vi "VIH - CHM Project - Write TOC File - Add LabVIEW Files.vi"(7 "Base Dir Path":path, 8 "error in":errorcluster, 9 "Project Files":T2, 11 "HTML in":string) -> (0 "error out":errorcluster, 3 "HTML out":string)   [LabVIEW 2014]
doc: "::: VI Helpeks :::\nCopyright (c) 2000-2026 Konstantin Shifershteyn. All rights reserved."
uses:
  _VIH HelpGen - Palette.llb/VIH HelpGen Typedef - Palette - Item Type Enum.ctl
panel:
  # "VI Helpeks\nCopyright (c) 2012-2026 Konstantin Shifershteyn"
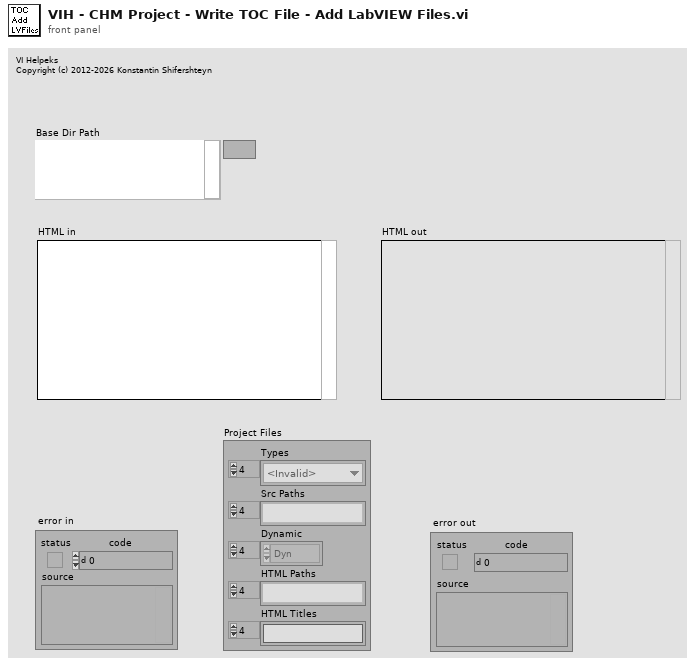
[diagram p1: front panel]
types:
  T1 = typedef "VIH HelpGen Typedef - Palette - Item Type Enum.ctl" = enum32{"<Invalid>", "<unknown>", "VI", "Menu", "LV Func", "Express VI", "Poly VI", "CTL", "HTML"}
  T2 = cluster{"Types":T1[], "Src Paths":path[], "Dynamic":enum16{"Dyn", "Stat", "Both"}[], "HTML Paths":path[], "HTML Titles":string[]}
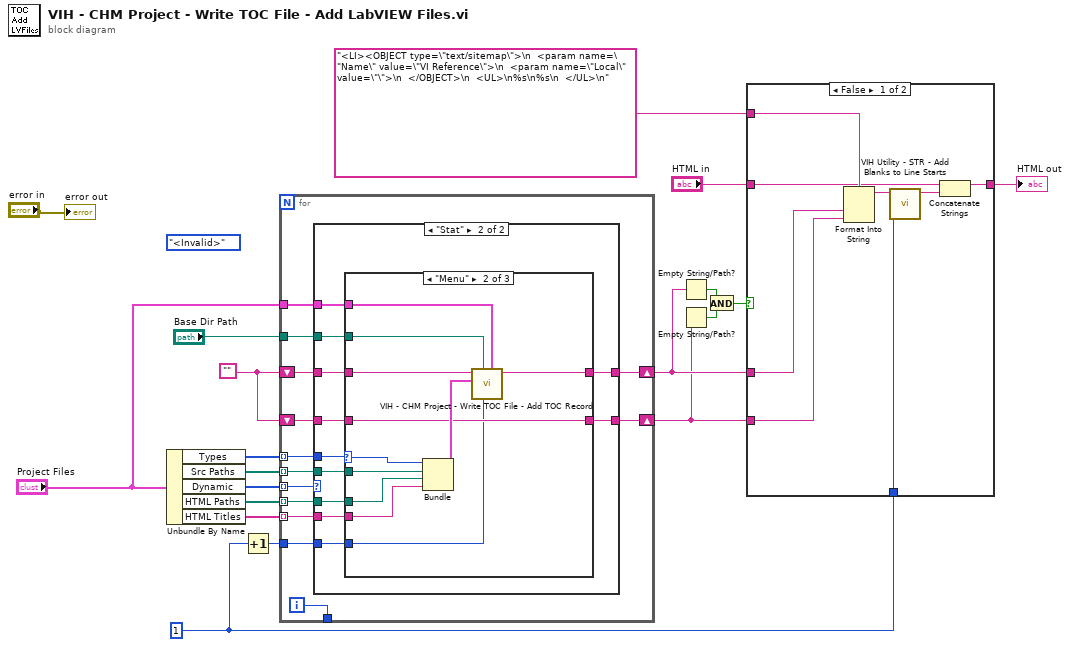
[diagram p0: block diagram]
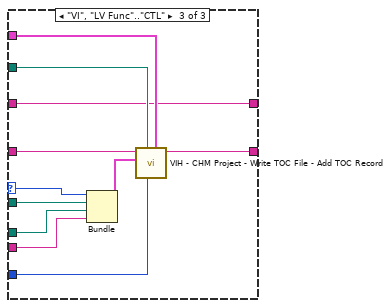
[diagram p5: hidden frame]
diagram:
  w2 = 1
  (unwired) VIH_HelpGen_Typedef_-_Palette_-_Item_Type_Enum."<Invalid>" ("Item/File Type")
  w11 = ""
  n1 = Unbundle By Name("Project Files") -> ("Types"=w17:T1[], "Src Paths"=w18:path[], "Dynamic"=w19:enum16{"Dyn", "Stat", "Both"}[], "HTML Paths"=w16:path[], "HTML Titles"=w14:string[])
  n2 = Increment(x=w2) -> (x+1=w1:i32)
  n3 = for {
    tunnel: w19 -> [w32] mode=indexing
    shift-right: [w29] -> w5
    shift-left: w11 -> [w31]
    tunnel: "Project Files" -> [w30]
    tunnel: w18 -> [w28] mode=indexing
    tunnel: w17 -> [w27] mode=indexing
    tunnel: w16 -> [w26] mode=indexing
    tunnel: "Base Dir Path" -> [w25]
    tunnel: w14 -> [w24] mode=indexing
    shift-right: [w22] -> w3
    shift-left: w11 -> [w23]
    tunnel: [w21] -> _
    tunnel: w1 -> [w20]
    i -> [w21]
    n4 = case shown="\"Stat\"" w32 {
      tunnel: w31 -> [w34 w45]
      tunnel: w30 -> [_ w44]
      tunnel: [w34 w43] -> w29
      tunnel: w28 -> [_ w41]
      tunnel: w27 -> [_ w38]
      tunnel: w26 -> [_ w40]
      tunnel: w25 -> [_ w42]
      tunnel: w24 -> [_ w39]
      tunnel: w23 -> [w33 w37]
      tunnel: [w33 w36] -> w22
      tunnel: w20 -> [_ w35]
      frame Default {
      }
      frame "Stat" {
        n5 = case shown="\"Menu\"" w38 {
          selector: w38 -> [_ w48 w59]
          tunnel: w45 -> [w47 w58 w62]
          tunnel: w44 -> [_ w57 w69]
          tunnel: [w47 w56 w62] -> w43
          tunnel: w42 -> [_ w55 w68]
          tunnel: w41 -> [_ w54 w67]
          tunnel: w40 -> [_ w53 w66]
          tunnel: w39 -> [_ w52 w65]
          tunnel: w37 -> [w46 w50 w63]
          tunnel: [w46 w50 w61] -> w36
          tunnel: w35 -> [_ w49 w60]
          frame "<Invalid>", "<unknown>", "HTML" {
          }
          frame "Menu" {
            n6 = Bundle("Item/File Type"=w48, w54, w53, w52) -> (w51:cluster{"Item/File Type":T1, path, path, string})  [unwired: 1 in]
            n7 = call "VIH - CHM Project - Write TOC File - Add TOC Record.vi"("Project Files"=w57, "Level"=w49, "Base Dir Path"=w55, "File Params"=w51, "HTML in"=w58) -> ("HTML out"=w56:string)  [unwired: 6 in]
          }
          frame "VI", "LV Func".."CTL" {
            n8 = Bundle("Item/File Type"=w59, w67, w66, w65) -> (w64:cluster{"Item/File Type":T1, path, path, string})  [unwired: 1 in]
            n9 = call "VIH - CHM Project - Write TOC File - Add TOC Record.vi"("Project Files"=w69, "Level"=w60, "Base Dir Path"=w68, "File Params"=w64, "HTML in"=w63) -> ("HTML out"=w61:string)  [unwired: 6 in]
          }
        }
      }
    }
  }
  n10 = Empty String/Path?(string/path=w5) -> (empty?=w10:bool)
  n11 = Empty String/Path?(string/path=w3) -> (empty?=w9:bool)
  n12 = And(x=w10, y=w9) -> (x .and. y?=w8:bool)
  n13 = case shown="False" w8 {
    tunnel: "HTML in" -> [w71 w78]
    tunnel: [w72 w78] -> w6
    tunnel: w5 -> [w77 _]
    tunnel: "<LI><OBJECT type=\"text/sitemap\">\n  <param name=\"Name\" value=\"VI Reference\">\n  <param name=\"Local\" value=\"\">\n  </OBJECT>\n  <UL>\n%s\n%s\n  </UL>\n" -> [w76 _]
    tunnel: w3 -> [w75 _]
    tunnel: w2 -> [w70 _]
    frame False {
      n14 = Format Into String(format string=w76, w77, w75) -> (resulting string=w74:string)  [unwired: 2 in, 1 out]
      n15 = call "VIH Utility - STR - Add Blanks to Line Starts.vi"("level"=w70, "String"=w74) -> ("String out"=w73:string)  [unwired: 9 in]
      n16 = Concatenate Strings(w71, w73) -> (w72:string)
    }
    frame True {
    }
  }
  "HTML out" <- w6
  "error out" <- "error in"
